vi "Write.vi"(0 "UCI_DllPath":path, 1 "Session_id":u32, 2 "Command":string="KEY:AT;", 3 "Timeout":u32=2000) -> (5 "ResultDescription":string)   [LabVIEW 2015]
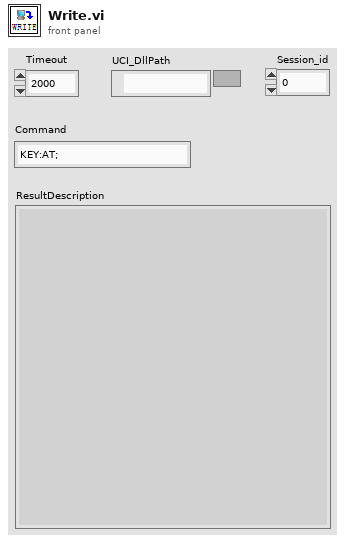
[diagram p1: front panel]
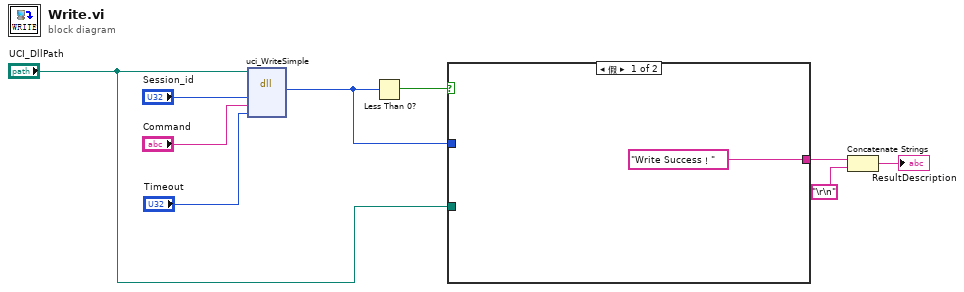
[diagram p0: block diagram]
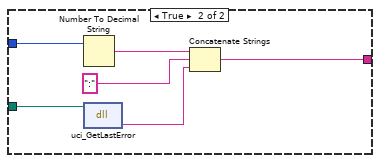
[diagram p2: hidden frame]
diagram:
  n1 = dll-call lib="E:/JL-Project/LabView-Project/ASCII/uci.dll" fn="uci_WriteSimple"(path in="UCI_DllPath", "session"="Session_id", "msg"="Command", "timeout"="Timeout") -> ("返回类型"=w6:i32)  [unwired: 5 in, 2 out]
  n2 = Less Than 0?(x=w6) -> (x < 0?=w7:bool)
  n3 = case shown="假" w7 {
    tunnel: w6 -> [_ w13]
    tunnel: "UCI_DllPath" -> [_ w12]
    tunnel: ["Write Success！" w11] -> w2
    frame False {
    }
    frame True {
      n4 = Number To Decimal String(number=w13) -> (decimal integer string=w14:string)  [unwired: 1 in]
      n5 = dll-call lib="E:/JL-Project/LabView-Project/ASCII/uci.dll" fn="uci_GetLastError"(path in=w12) -> ("返回类型"=w16:string)  [unwired: 2 in, 2 out]
      n6 = Concatenate Strings(w14, ":" ("字符串"), w16) -> (w11:string)
    }
  }
  n7 = Concatenate Strings(w2, "\r\n") -> (→"ResultDescription":string)
